vi "MRC Testing.vi"() -> ()   [LabVIEW 2026]
uses:
  <vilib>/Rock Robotics/WPI/DriverStation/WPI_DriverStationAllianceInfo.ctl
  <vilib>/Rock Robotics/WPI/DriverStation/WPI_DriverStationPositionInfo.ctl
  <vilib>/Rock Robotics/Network Tables/NT Write String Array.vi
  <vilib>/MRC/MrcLib.lvlib
panel:
  out "Array":cluster{"currentOpMode":u64, "Enabled":bool}[](array[cluster]) {"currentOpMode" format="%.0x"}
  in  "stop":bool
  in  "auto names":string[](array[string])=["Auto 0", "Auto foo"]
  out "Enabled":bool
  out "RobotMode":u8
  out "OutputsEnabled?":bool
  out "details":T1
  out "Match Time(s)":sgl
  out "currentOpMode":u64 format="%.0x"
  out "Alliance":cluster{"Color":T2, "Position":T3}
  out "input voltage (V)":dbl
  out "Game Specific Data":string
  out "Team Number":string
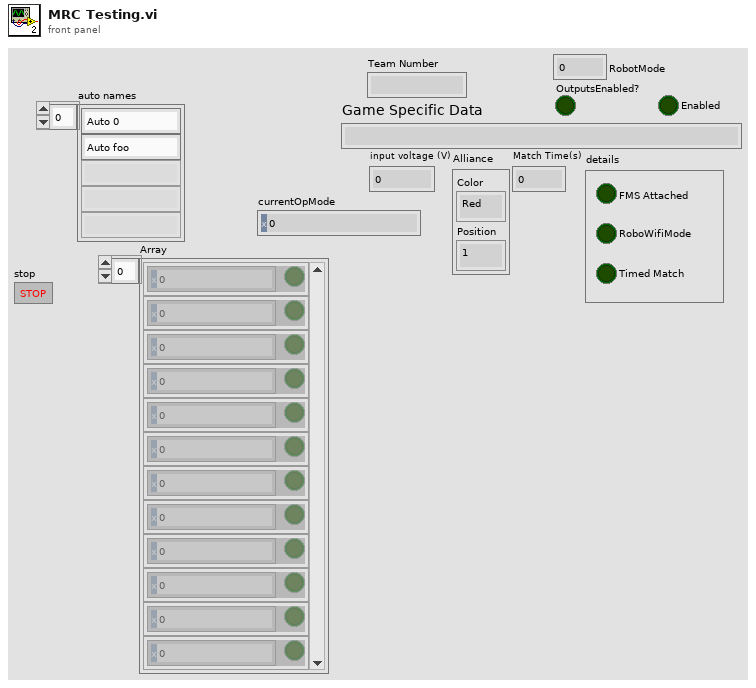
[diagram p1: front panel]
types:
  T1 = cluster{"FMS Attached":bool, "RoboWifiMode":bool, "Timed Match":bool}
  T2 = typedef "WPI_DriverStationAllianceInfo.ctl" = enum16{"Red", "Blue", "Invalid"}
  T3 = typedef "WPI_DriverStationPositionInfo.ctl" = enum16{"1", "2", "3"}
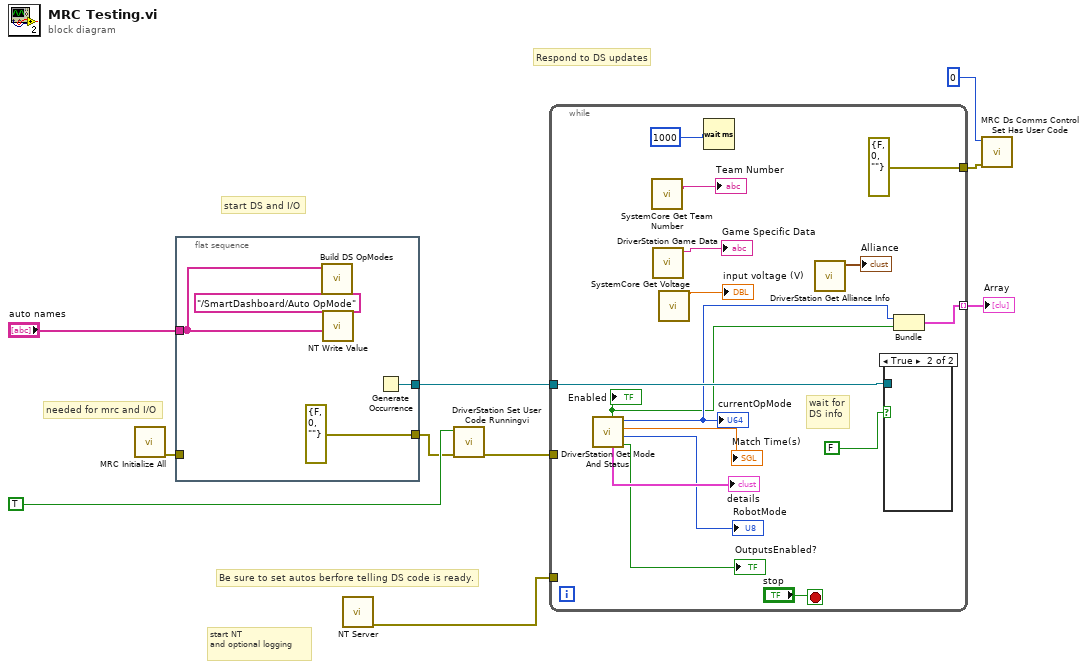
[diagram p0: block diagram]
diagram:
  # "Respond to DS updates"
  # "start DS and I/O"
  # "start NT\nand optional logging"
  # "needed for mrc and I/O"
  # "Be sure to set autos berfore telling DS code is ready."
  n1 = call <vilib>:"MRC Initialize All.vi"() -> ("error out"=w9:errorcluster)  [unwired: 11 in]
  n2 = flat-sequence {
    tunnel: [errorcluster {"status"=FALSE, "code"=0, "source"=""} ("error in (no error)")] -> w8
    tunnel: w9 -> [_]
    tunnel: [w12] -> w7
    tunnel: "auto names" -> [w11]
    frame #0 {
      n3 = call <vilib>:"Build DS OpModes.vi"("auto names"=w11) -> ()  [unwired: 11 in]
      n4 = call-poly <vilib>:"NT Write Value.vi"("value"=w11, "name"="/SmartDashboard/Auto OpMode") -> ()  [unwired: 9 in, 1 out]
      n5 = Generate Occurrence() -> (w12:refnum<k4>)
    }
  }
  n6 = call <vilib>:"NT Server.vi"() -> ("error out"=w5:errorcluster)  [unwired: 11 in]
  n7 = call <vilib>:"DriverStation Set User Code Runningvi.vi"("error in (no error)"=w8, "code ready for enable"=TRUE) -> ("error out"=w6:errorcluster)  [unwired: 9 in]
  n8 = while {
    tunnel: w6 -> [_]
    tunnel: w7 -> [w21]
    tunnel: w5 -> [_]
    tunnel: [w16] -> w3 mode=indexing
    tunnel: [errorcluster {"status"=FALSE, "code"=0, "source"=""} ("error in (no error)")] -> w2
    stop <- "stop" stop-if-true
    # "wait for\nDS info"
    n9 = call <vilib>:"DriverStation Get Mode And Status.vi"() -> ("OutputsEnabled?"=→"OutputsEnabled?":bool, "RobotMode"=→"RobotMode":u8, "Match Time(s)"=→"Match Time(s)":sgl, "currentOpMode"=w18:u64, "details"=→"details":T1, "Enabled"=w17:bool)  [unwired: 6 in]
    "currentOpMode" <- w18
    "Enabled" <- w17
    n10 = call <vilib>:"SystemCore Get Team Number.vi"() -> ("Team Number"=→"Team Number":string)  [unwired: 14 in, 1 out]
    n11 = call <vilib>:"DriverStation Game Data.vi"() -> ("Game Specific Data"=→"Game Specific Data":string)  [unwired: 11 in]
    n12 = call <vilib>:"SystemCore Get Voltage.vi"() -> ("input voltage (V)"=→"input voltage (V)":dbl)  [unwired: 14 in, 1 out]
    n13 = Wait (ms)(milliseconds to wait=u32 1000) -> ()  [unwired: 1 out]
    n14 = call <vilib>:"DriverStation Get Alliance Info.vi"() -> ("Alliance"=→"Alliance":cluster{"Color":T2, "Position":T3})  [unwired: 7 in, 4 out]
    n15 = case shown="True" FALSE {
      tunnel: w21 -> [_ _]
      frame False {
      }
      frame True {
      }
    }
    n16 = Bundle("currentOpMode"=w18, "Enabled"=w17) -> (w16:cluster{"currentOpMode":u64, "Enabled":bool})  [unwired: 1 in]
  }
  "Array" <- w3
  n17 = call <vilib>:"MRC Ds Comms Control Set Has User Code.vi"("error in (no error)"=w2, "hasUserCode"=u8 0) -> ()  [unwired: 9 in, 1 out]
